vi "RemoteVI Fixture Layout.vi"(0 "Panel":refnum<vi>, 5 "Origin":cluster{"Horizontal":i32, "Vertical":i32}, 11 "error in":errorcluster) -> (4 "layout":string, 15 "error out":errorcluster)   [LabVIEW 2020]
doc: "Event-log helper of RemoteVI Fixture.vi. Builds the layout lines of the log: for every control on Panel whose label is one of Switch, Button, Number, Text, Mode, Tab, Graph, List, Ask, Open, Stop one line layout TAB label TAB x y w h LF, the control's body rectangle (Position and Bounds, without the label) in panel-image coordinates, that is minus the window Origin. Other controls are skipped. Errors of the property reads go to error out."
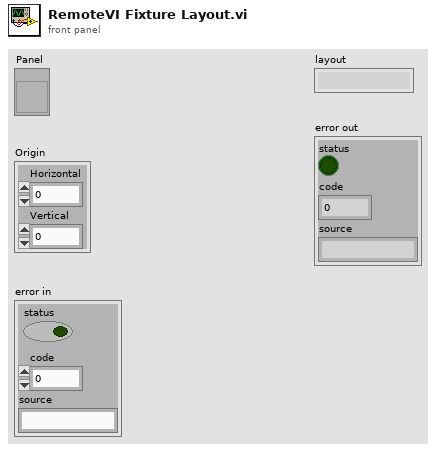
[diagram p1: front panel]
types:
  T1 = typedef "LVPositionTypeDef.ctl" = cluster{"Left":i32, "Top":i32}
  T2 = typedef "LVBoundsTypeDef.ctl" = cluster{"Width":u32, "Height":u32}
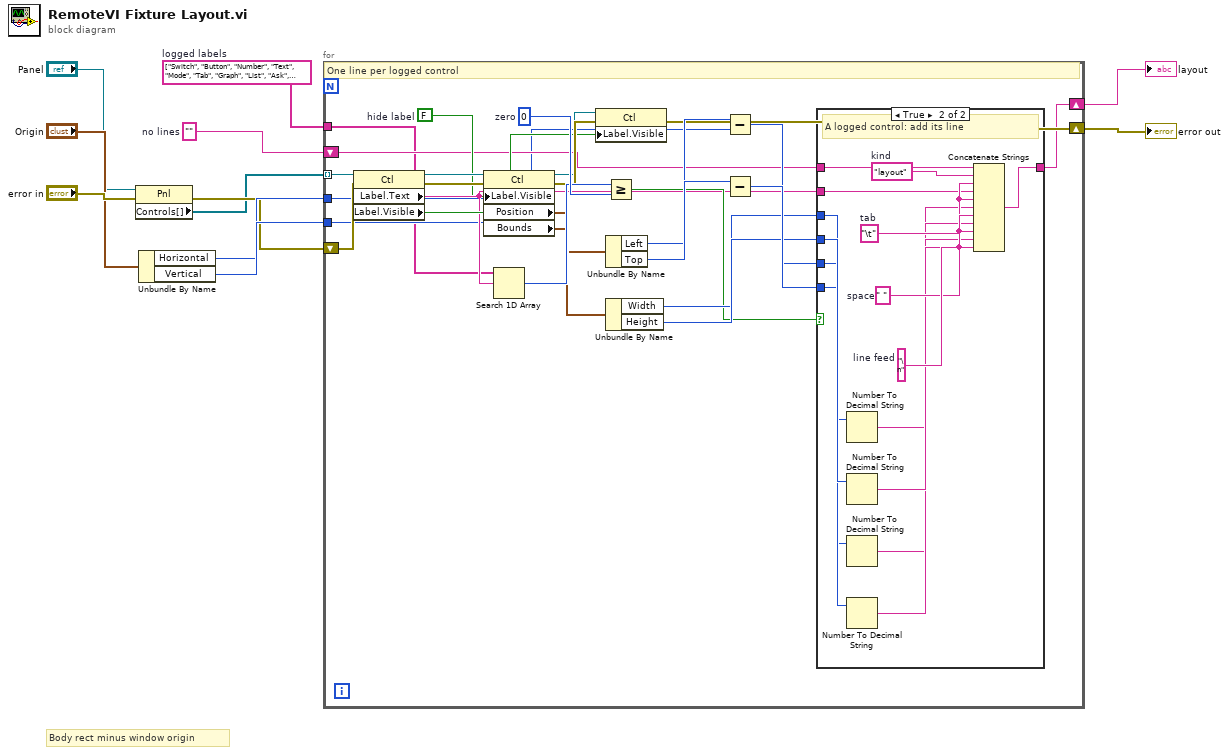
[diagram p0: block diagram]
diagram:
  w7 = ""  # no lines
  w6 = string[] ["Switch", "Button", "Number", "Text", "Mode", "Tab", "Graph", "List", "Ask", "Open", "Stop"]  # logged labels
  # "Body rect minus window origin"
  n1 = property class="Pnl"(reference="Panel", error in="error in") -> (error out=w5:errorcluster, "Controls[]"=w4:refnum<vi>[])  [unwired: 1 out]
  n2 = Unbundle By Name("Origin") -> ("Horizontal"=w8:i32, "Vertical"=w9:i32)
  n3 = for {
    tunnel: w6 -> [w13]
    shift-right: [w17] -> w10
    shift-left: w7 -> [w16]
    tunnel: w4 -> [w12] mode=indexing
    tunnel: w8 -> [w14]
    tunnel: w9 -> [w15]
    shift-right: [w19] -> w11
    shift-left: w5 -> [w18]
    w30 = 0  # zero
    w20 = FALSE  # hide label
    # "One line per logged control"
    n4 = property class="Ctl"(reference=w12, error in=w18) -> (reference out=w23:refnum<vi>, error out=w24:errorcluster, "Label.Text"=w21:string, "Label.Visible"=w22:bool)
    n5 = property class="Ctl"(reference=w23, error in=w24, "Label.Visible"=w20) -> (reference out=w27:refnum<vi>, error out=w28:errorcluster, "Position"=w25:T1, "Bounds"=w26:T2)
    n6 = Search 1D Array(1D array=w13, element=w21) -> (index of element=w29:i32)  [unwired: 1 in]
    n7 = property class="Ctl"(reference=w27, error in=w28, "Label.Visible"=w22) -> (error out=w19:errorcluster)  [unwired: 1 out]
    n8 = Greater Or Equal?(x=w29, y=w30) -> (x >= y?=w31:bool)
    n9 = Unbundle By Name(w25) -> ("Left"=w32:i32, "Top"=w33:i32)
    n10 = Unbundle By Name(w26) -> ("Width"=w34:u32, "Height"=w35:u32)
    n11 = Subtract(x=w32, y=w14) -> (x-y=w36:i32)
    n12 = Subtract(x=w33, y=w15) -> (x-y=w37:i32)
    n13 = case shown="True" w31 {
      tunnel: w16 -> [w38 w39]
      tunnel: w21 -> [_ w40]
      tunnel: w34 -> [_ w43]
      tunnel: w35 -> [_ w44]
      tunnel: w36 -> [_ w41]
      tunnel: w37 -> [_ w42]
      tunnel: [w38 w53] -> w17
      frame False {
        # "Any other control: skip"
      }
      frame True {
        w52 = "\n"  # line feed
        w51 = " "  # space
        w50 = "\t"  # tab
        w49 = "layout"  # kind
        # "A logged control: add its line"
        n14 = Number To Decimal String(number=w43) -> (decimal integer string=w47:string)  [unwired: 1 in]
        n15 = Number To Decimal String(number=w44) -> (decimal integer string=w48:string)  [unwired: 1 in]
        n16 = Number To Decimal String(number=w41) -> (decimal integer string=w45:string)  [unwired: 1 in]
        n17 = Number To Decimal String(number=w42) -> (decimal integer string=w46:string)  [unwired: 1 in]
        n18 = Concatenate Strings(w39, w49, w50, w40, w50, w45, w51, w46, w51, w47, w51, w48, w52) -> (w53:string)
      }
    }
  }
  "layout" <- w10
  "error out" <- w11
